vi "query SCPI command.vi"(8 "error in (no error)":errorcluster, 9 "Read Buffer Length":u32, 10 "SCPI Command":string, 11 "LTE in":refnum<class "LTE.lvclass">) -> (0 "error out":errorcluster, 2 "Read Buffer String":string, 3 "LTE out":refnum<class "LTE.lvclass">)   [LabVIEW 2023, in "ANRITSU Call Box.lvlib" / "LTE.lvclass"]
uses:
  LTE.lvclass
  LTE.lvclass/LTE.ctl
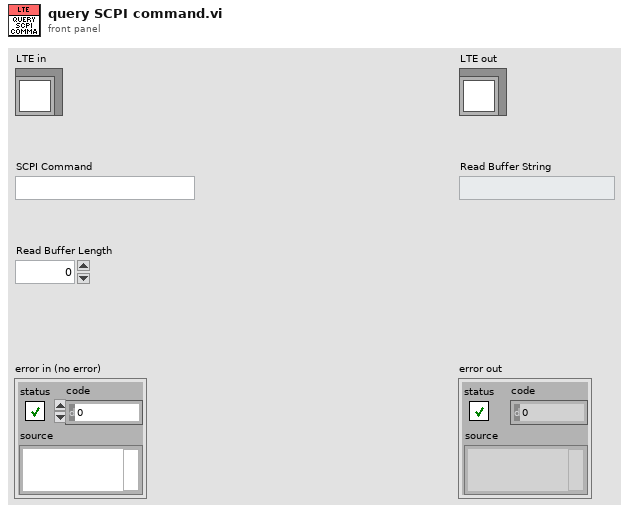
[diagram p1: front panel]
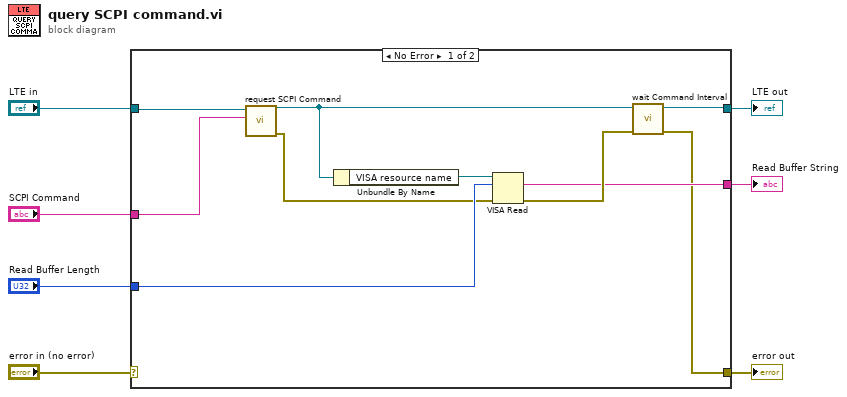
[diagram p0: block diagram]
diagram:
  n1 = case shown="No Error" "error in (no error)" {
    selector: "error in (no error)" -> [_ w19]
    tunnel: [w8 w19] -> w6
    tunnel: [w15 w18] -> w4
    tunnel: "LTE in" -> [w17 w18]
    tunnel: "SCPI Command" -> [w16 _]
    tunnel: "Read Buffer Length" -> [w12 _]
    tunnel: [w9 _] -> w1
    frame No Error {
      n2 = call "request SCPI Command.vi"("SCPI Command"=w16, "LTE in"=w17) -> ("error out"=w11:errorcluster, "LTE out"=w14:refnum<class "LTE.lvclass">)  [unwired: 8 in]
      n3 = Unbundle By Name(w14) -> ("VISA resource name"=w13:refnum<visa-resource-name>)
      n4 = VISA Read(VISA resource name=w13, byte count=w12, error in (no error)=w11) -> (read buffer=w9:string, error out=w10:errorcluster)  [unwired: 2 out]
      n5 = call "wait Command Interval.vi"("error in (no error)"=w10, "LTE in"=w14) -> ("error out"=w8:errorcluster, "LTE out"=w15:refnum<class "LTE.lvclass">)  [unwired: 8 in]
    }
    frame Error {
    }
  }
  "error out" <- w6
  "LTE out" <- w4
  "Read Buffer String" <- w1
